vi "Add Flag.vi"(11 "数组IN":string[](array[string])) -> (3 "数组":string[](array[string]), 4 "table1":string)   [LabVIEW 2025]
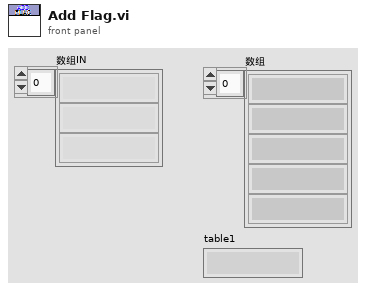
[diagram p1: front panel]
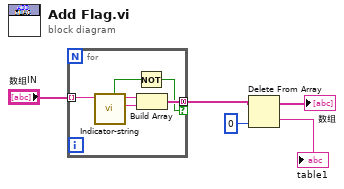
[diagram p0: block diagram]
diagram:
  n1 = for {
    tunnel: "数组IN" -> [w10] mode=indexing
    tunnel: [w11] -> w4 mode=concatenating if=w6
    n2 = call "Indicator-string.vi"("字符串"=w10) -> ("退表名"=w8:string, "进表名"=w9:string, "为空？"=w7:bool)  [unwired: 8 in]
    n3 = Not(x=w7) -> (.not. x?=w6:bool)
    n4 = Build Array(w9, w8) -> (w11:string[])
  }
  n5 = Delete From Array(array=w4, index=0 ("索引")) -> (deleted portion=→"table1":string, array with subset deleted=→"数组":string[])  [unwired: 1 in]
